vi "Begin Step.vi"(8 "error in":errorcluster, 11 "Sequence Executor in":refnum<class "Sequence Executor.lvclass">) -> (0 "error out":errorcluster, 3 "Sequence Executor out":refnum<class "Sequence Executor.lvclass">)   [LabVIEW 2026, in "Sequence Executor.lvclass"]
doc: "PRIVATE. Begins Results[Step Index]: result RUNNING, Phase Settling, Step Start ms -1, Dwell Start ms 0, sends Apply Setpoints Msg with the step's setpoints to the rig, then refreshes the displays (Status RUNNING)."
uses:
  Sequence Executor.lvclass
  Sequence Executor.lvclass/Sequence Executor.ctl
  Rig Messages/Apply Setpoints Msg/Apply Setpoints Msg.lvclass/Apply Setpoints Msg.ctl
  <vilib>/ActorFramework/Message Enqueuer/Message Enqueuer.lvclass/Message Enqueuer.ctl
  <vilib>/ActorFramework/Message Enqueuer/Enqueue.vi
  Rig Messages/Apply Setpoints Msg/Apply Setpoints Msg.lvclass
  <vilib>/ActorFramework/Message Priority Queue/Priority Enqueue.vi
  <vilib>/ActorFramework/Message Enqueuer/Message Enqueuer.lvclass
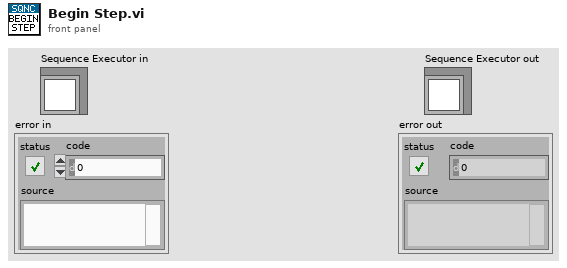
[diagram p1: front panel]
types:
  T1 = typedef "Sequence File.ctl" = cluster{"sequence_id":string, "description":string, "rig_config":string, "steps":T2[]}
  T2 = typedef "Step Config.ctl" = cluster{"step_no":i32, "step_name":string, "command_type":string, "setpoints":T3[], "conditions":T4[], "dwell_time_ms":i32, "timeout_ms":i32, "expected_result":string}
  T3 = typedef "Channel Value.ctl" = cluster{"channel":string, "value":dbl}
  T4 = typedef "Condition.ctl" = cluster{"channel":string, "target":dbl, "tolerance":dbl}
  T5 = typedef "Step Result.ctl" = cluster{"step_no":i32, "step_name":string, "result":string, "reason":string, "measured":dbl, "target":dbl, "duration_ms":dbl}
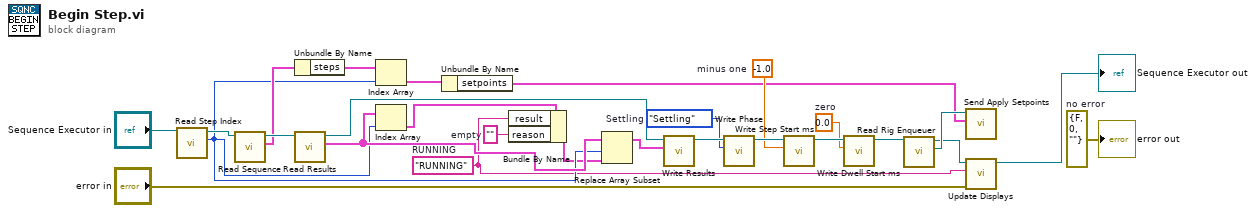
[diagram p0: block diagram]
diagram:
  w9 = 0.0  # zero
  w11 = -1.0  # minus one
  w13 = enum16{"Idle", "Settling", "Dwell", "Complete"}."Settling"  # Settling
  w21 = ""  # empty
  w4 = "RUNNING"  # RUNNING
  w1 = errorcluster {"status"=FALSE, "code"=0, "source"=""}  # no error
  n1 = call "Read Step Index.vi"("Sequence Executor in"="Sequence Executor in") -> ("Step Index"=w18:i32, "Sequence Executor out"=w26:refnum<class "Sequence Executor.lvclass">)  [unwired: 8 in, 1 out]
  n2 = call "Read Sequence.vi"("Sequence Executor in"=w26) -> ("Sequence File"=w24:T1, "Sequence Executor out"=w25:refnum<class "Sequence Executor.lvclass">)  [unwired: 8 in, 1 out]
  n3 = Unbundle By Name(w24) -> ("steps"=w23:T2[])
  n4 = call "Read Results.vi"("Sequence Executor in"=w25) -> ("Results"=w19:T5[], "Sequence Executor out"=w16:refnum<class "Sequence Executor.lvclass">)  [unwired: 8 in, 1 out]
  n5 = Index Array(array=w23, index=w18) -> (element=w22:T2)
  n6 = Index Array(array=w19, index=w18) -> (element=w20:T5)
  n7 = Unbundle By Name(w22) -> ("setpoints"=w6:T3[])
  n8 = Bundle By Name(cluster=w20, "result"=w4, "reason"=w21) -> (w17:T5)
  n9 = Replace Array Subset(array=w19, new element=w17, index=w18) -> (w15:T5[])
  n10 = call "Write Results.vi"("Results"=w15, "Sequence Executor in"=w16) -> ("Sequence Executor out"=w14:refnum<class "Sequence Executor.lvclass">)  [unwired: 8 in, 1 out]
  n11 = call "Write Phase.vi"("Step Phase"=w13, "Sequence Executor in"=w14) -> ("Sequence Executor out"=w12:refnum<class "Sequence Executor.lvclass">)  [unwired: 8 in, 1 out]
  n12 = call "Write Step Start ms.vi"("Step Start ms"=w11, "Sequence Executor in"=w12) -> ("Sequence Executor out"=w10:refnum<class "Sequence Executor.lvclass">)  [unwired: 8 in, 1 out]
  n13 = call "Write Dwell Start ms.vi"("Dwell Start ms"=w9, "Sequence Executor in"=w10) -> ("Sequence Executor out"=w8:refnum<class "Sequence Executor.lvclass">)  [unwired: 8 in, 1 out]
  n14 = call "Read Rig Enqueuer.vi"("Sequence Executor in"=w8) -> ("Actor Framework:Message Enqueuer"=w7:refnum<class "Message Enqueuer.lvclass">, "Sequence Executor out"=w5:refnum<class "Sequence Executor.lvclass">)  [unwired: 8 in, 1 out]
  n15 = call "Send Apply Setpoints.vi"("setpoints"=w6, "Message Enqueuer"=w7) -> ()  [unwired: 8 in, 2 out]
  n16 = call "Update Displays.vi"("error in"="error in", "Status"=w4, "Sequence Executor in"=w5) -> ("Sequence Executor out"=→"Sequence Executor out":refnum<class "Sequence Executor.lvclass">)  [unwired: 7 in, 1 out]
  "error out" <- w1
